vi "Test_C_W12_W13_Quick.vi"() -> ()   [LabVIEW 2021]
uses:
  CANsub_C.lvlib
  C_Decode_Result.ctl
panel:
  out "size data":i32
  out "id":u32[](array[numeric]) format="%.0x"
  out "data len":u8[](array[numeric])
  out "dlc":u8[](array[numeric])
  out "size hdlc":i32
  out "size ping":i32
  out "data":u8[](array[numeric])
  out "size ws":i32
  out "result":T1
  # "Expected values when run."
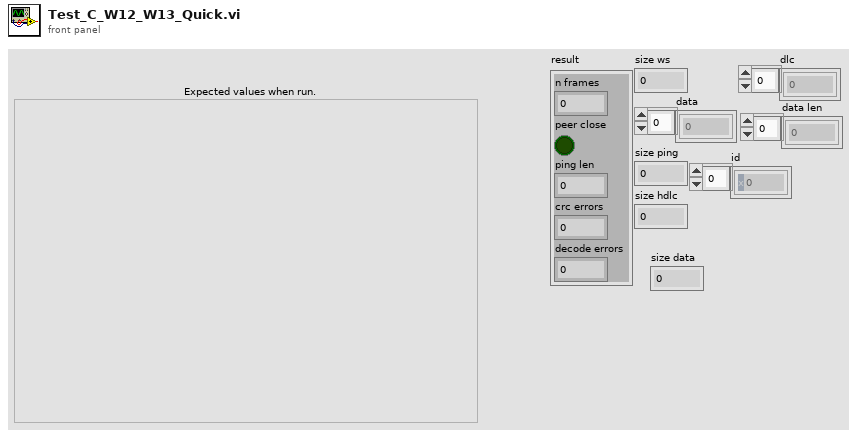
[diagram p1: front panel]
types:
  T1 = typedef "CANsub_C.lvlib/C_Decode_Result.ctl" = cluster{"n frames":i32, "peer close":bool, "ping len":i32, "crc errors":u32, "decode errors":i32}
  T2 = typedef "CANsub_C.lvlib/C_RX_Buffers.ctl" = cluster{"t_dev":dbl[], "ws":u8[], "id":u32[], "flags":u16[], "hdlc":u8[], "dlc":u8[], "data len":u8[], "data":u8[], "ping":u8[]}
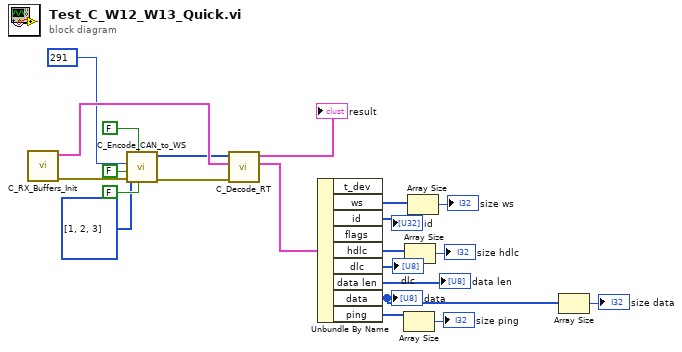
[diagram p0: block diagram]
diagram:
  n1 = call "C_RX_Buffers_Init.vi"() -> ("error out"=w21:errorcluster, "buffers"=w19:T2)  [unwired: 8 in, 2 out]
  n2 = call "C_Encode_CAN_to_WS.vi"("brs"=FALSE, "ide"=FALSE, "error in (no error)"=w21, "fdf"=FALSE, "id"=u32 291, "data"=u8[] [1, 2, 3]) -> ("error out"=w20:errorcluster, "ws frame"=w13:u8[])  [unwired: 4 in]
  n3 = call "C_Decode_RT.vi"("error in (no error)"=w20, "buffers in"=w19, "bytes in"=w13) -> ("buffers out"=w22:T2, "result"=→"result":T1)  [unwired: 6 in, 1 out]
  n4 = Unbundle By Name(w22) -> ("ws"=w11:u8[], "id"=→"id":u32[], "hdlc"=w7:u8[], "dlc"=→"dlc":u8[], "data len"=→"data len":u8[], "data"=w2:u8[], "ping"=w9:u8[])  [unwired: 2 out]
  "data" <- w2
  n5 = Array Size(array=w9) -> (size(s)=→"size ping":i32)
  n6 = Array Size(array=w7) -> (size(s)=→"size hdlc":i32)
  n7 = Array Size(array=w11) -> (size(s)=→"size ws":i32)
  n8 = Array Size(array=w2) -> (size(s)=→"size data":i32)
